vi "PicoScope2000aSetEts.vi"(7 "ETS Mode":u32(ring) items=["PS3000A_ETS_OFF", "PS3000A_ETS_FAST", "PS3000A_ETS_SLOW"], 8 "error in (no error)":errorcluster, 9 "etsInterleave":i16, 10 "etsCycles":i16, 11 "handle in":i16) -> (0 "error out":errorcluster, 3 "handle out":i16, 4 "sampleTimePicoseconds":i32)   [LabVIEW 2009]
doc: "Calls SetETS"
uses:
  ps2000a.dll
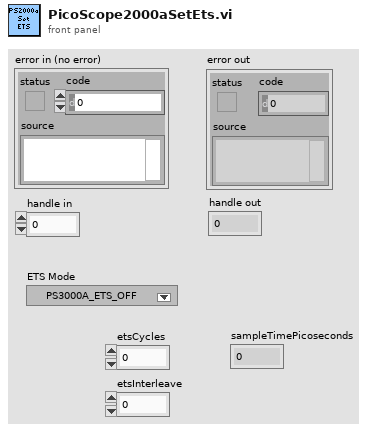
[diagram p1: front panel]
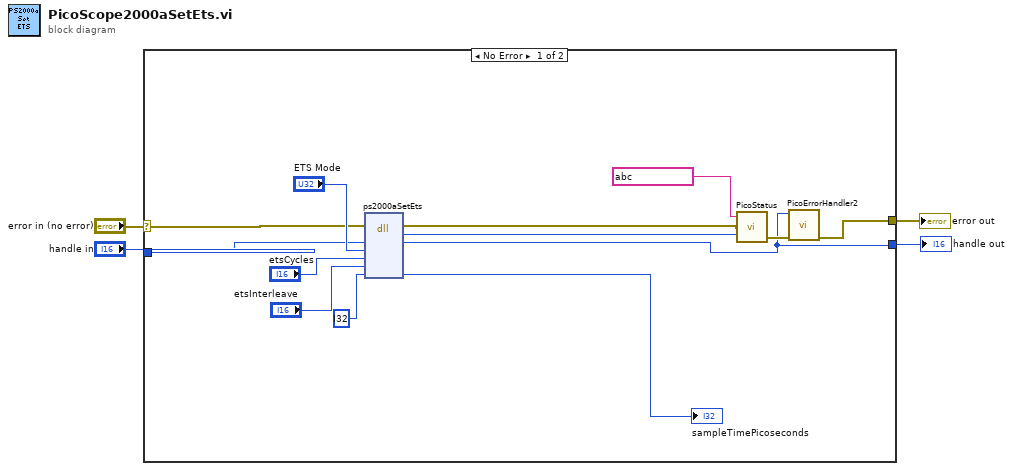
[diagram p0: block diagram]
diagram:
  n1 = case shown="No Error" "error in (no error)" {
    selector: "error in (no error)" -> [w13 w19]
    tunnel: [w16 w19] -> w2
    tunnel: "handle in" -> [w12 w18]
    tunnel: [w8 w18] -> w3
    frame #0 {
      n2 = dll-call lib="ps2000a.dll" fn="ps2000aSetEts" ("ps3000.dll:_ps3000_open_unit@0")(error in=w13, "handle"=w12, "mode"="ETS Mode", "etsCycles"="etsCycles", "etsInterleave"="etsInterleave", "sampleTimePicoseconds"=i32 ?) -> (error out=w10:errorcluster, "PICO_STATUS"=w9:u32, "handle"=w8:i16, "sampleTimePicoseconds"=→"sampleTimePicoseconds":i32)  [unwired: 5 in, 1 out]
      n3 = call "PicoStatus.vi"("PICO STATUS"=w9, "error in"=w10, "source"=string ?) -> ("error out"=w17:errorcluster)
      n4 = call "PicoErrorHandler2.vi"("error in (no error)"=w17, "handle In"=w8) -> ("error out"=w16:errorcluster)  [unwired: 9 in]
    }
    frame #1 {
    }
  }
  "error out" <- w2
  "handle out" <- w3
